vi "Create StaticVIRefnum Job.vi"(5 "Job.StaticVIRef in":refnum<class "Job.StaticVIRef.lvclass">, 6 "JobReport type":refnum<class "JobReport.lvclass">, 7 "Job Name":string, 8 "error in (no error)":errorcluster, 9 "Output Terminal Name (stdout)":string="stdout", 10 "Input Terminal Name (stdin)":string="stdin", 11 "Static VI Refnum":refnum<vi>) -> (0 "error out":errorcluster, 3 "Job.StaticVIRef out":refnum<class "Job.StaticVIRef.lvclass">)   [LabVIEW 2013, in "openCronJob.lvlib" / "Job.StaticVIRef.lvclass"]
uses:
  Job.StaticVIRef.lvclass
  JobReport/JobReport.lvclass
  Job.StaticVIRef.lvclass/Job.StaticVIRef.ctl
  Job/Job.lvclass
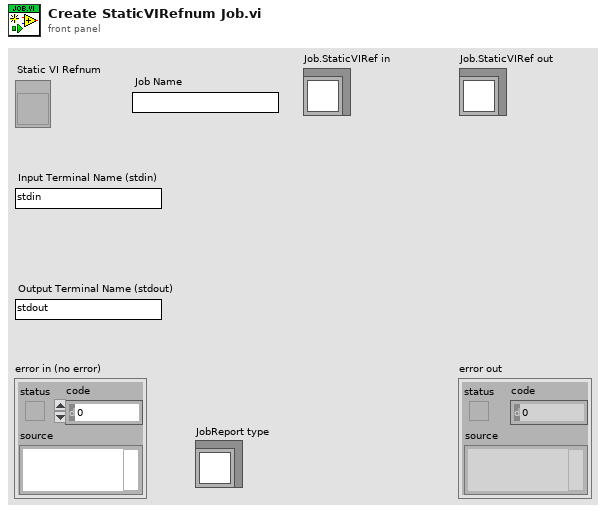
[diagram p1: front panel]
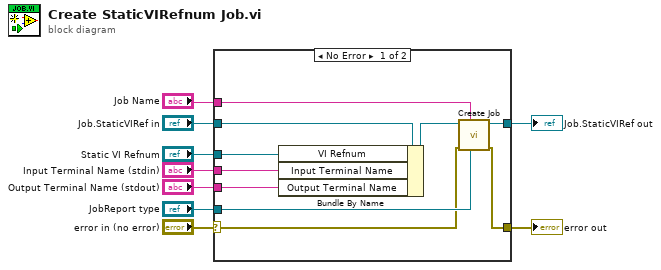
[diagram p0: block diagram]
diagram:
  n1 = case shown="No Error" "error in (no error)" {
    selector: "error in (no error)" -> [w11 w21]
    tunnel: [w10 w21] -> w8
    tunnel: [w14 w20] -> w6
    tunnel: "Job.StaticVIRef in" -> [w18 w20]
    tunnel: "Static VI Refnum" -> [w19 _]
    tunnel: "Input Terminal Name (stdin)" -> [w17 _]
    tunnel: "Output Terminal Name (stdout)" -> [w16 _]
    tunnel: "Job Name" -> [w13 _]
    tunnel: "JobReport type" -> [w12 _]
    frame No Error {
      n2 = Bundle By Name(cluster=w18, "VI Refnum"=w19, "Input Terminal Name"=w17, "Output Terminal Name"=w16) -> (w15:refnum<class "Job.StaticVIRef.lvclass">)
      n3 = call "Create Job.vi"("JobReport type"=w12, "Job Name"=w13, "error in (no error)"=w11, "Job in"=w15) -> ("error out"=w10:errorcluster, "Job"=w14:refnum<class "Job.StaticVIRef.lvclass">)  [unwired: 6 in]
    }
    frame Error {
    }
  }
  "error out" <- w8
  "Job.StaticVIRef out" <- w6
